vi "VHistFile - Read-Write CDB Log File.vi"(4 "time range to read":cluster{"t1":dbl, "t2":dbl} {"t2" format="%<%H:%M:%S%2u\n%d/%m/%Y>T"; "t1" format="%<%H:%M:%S%2u\n%d/%m/%Y>T"}, 5 "file params":T1={"path pattern"=enum."Y\\M\\D\\Tag.ext", "file extension (.bin)"=".bin"}, 6 "operation":enum16{"nop", "read", "write", "retrieve"}(ring), 7 "log directory":path=path "DataLog", 8 "error in":errorcluster, 9 "history data in":cdb[](array[numeric]) format="%.2f", 10 "time stamps in":dbl[](array[numeric]) format="%<%H:%M:%S%2u\n%d/%m/%Y>T", 11 "file tag":string) -> (0 "error out":errorcluster, 1 "history data out":cdb[](array[numeric]) format="%.2f", 2 "time stamps out":dbl[](array[numeric]) format="%<%H:%M:%S%2u\n%d/%m/%Y>T")   [LabVIEW 2021]
doc: "The VI writes and reads log files intended to store historical data that have <b>CDB Scalar</b> datatype.\n\nA log file record consists of a time stamp and respective data value. VI maintains a separate file for every date; i.e. data values stored in a log file have time stamps belonging to the same date. In addition, VI supports a few file path patterns that define a structure of subdirectories within a basic log directory to store log files and file name format.\n\nVI performs all operations to maintain this file arrangement transparently for applications. An application has only to specify a <b>file tag</b> that is used as a unique data identifier and, optionally, file path pattern and a file name extension.\n\nWhen VI writes historic data, it saves data values and time stamps to the respective file(s). If a file exists, VI appends new records to the end of file. If a file does not exist, VI automatically creates it along with a subdirectory structure it should reside. If an input data set contains values belonging to different dates, VI stores every value to an appropriate location.\n\nWhen VI reads historic data, it automatically retrieves data with time stamps belonging to the specified time range even if required data are stored in several files and, probably, directories. The only required thing is to provide the same file parameters for reading as were used for writing; i.e. file tag, basic log directory, file path pattern and file extension.\n\n::: CalcExpress Toolkit :::\nCopyright (c) 2000-2026 Konstantin Shifershteyn. All rights reserved."
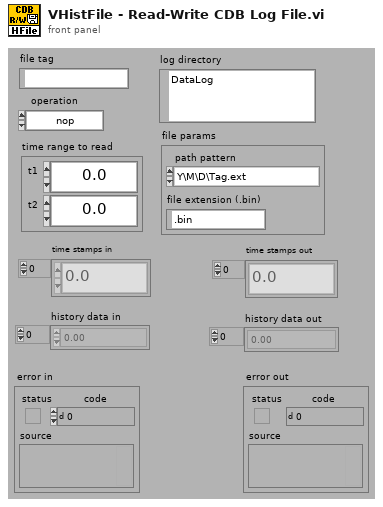
[diagram p1: front panel]
types:
  T1 = cluster{"path pattern":enum32{"Y\\M\\D\\Tag.ext", "Y\\M\\D\\Tag [Y-M-D].ext", "Y-M-D\\Tag.ext", "Y-M-D\\Tag [Y-M-D].ext", "Tag [Y-M-D].ext"}, "file extension (.bin)":string}
  T2 = enum32{"Y\\M\\D\\Tag.ext", "Y\\M\\D\\Tag [Y-M-D].ext", "Y-M-D\\Tag.ext", "Y-M-D\\Tag [Y-M-D].ext", "Tag [Y-M-D].ext"}
  T3 = enum16{"read/write", "read-only", "write-only", "write-only (truncate)"}
  T4 = enum16{"big-endian, network order", "native, host order", "little-endian"}
  T5 = enum16{"deny read/write", "deny write-only", "deny none"}
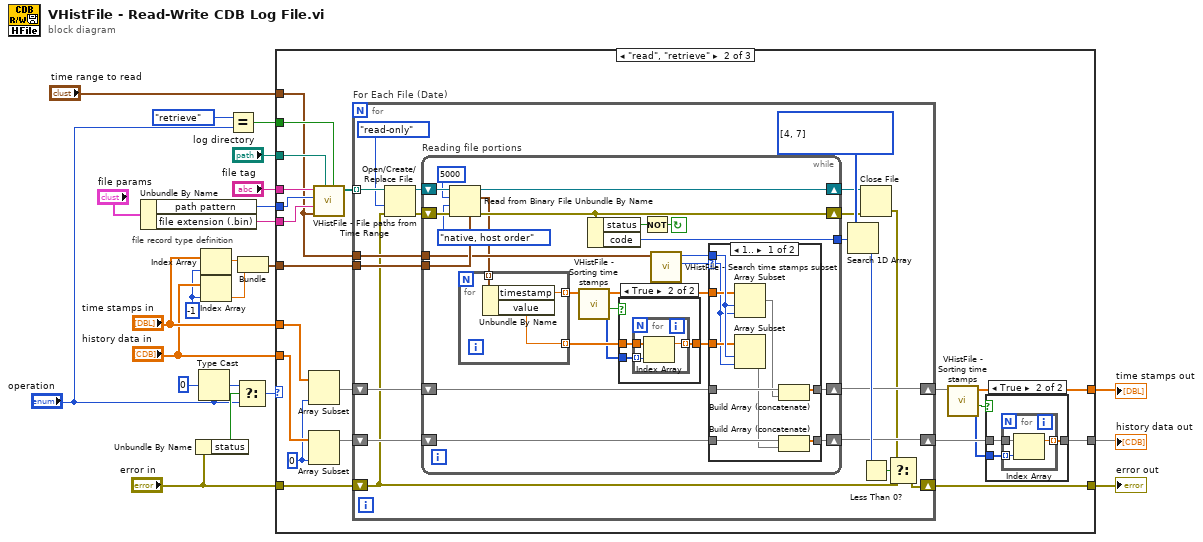
[diagram p0: block diagram]
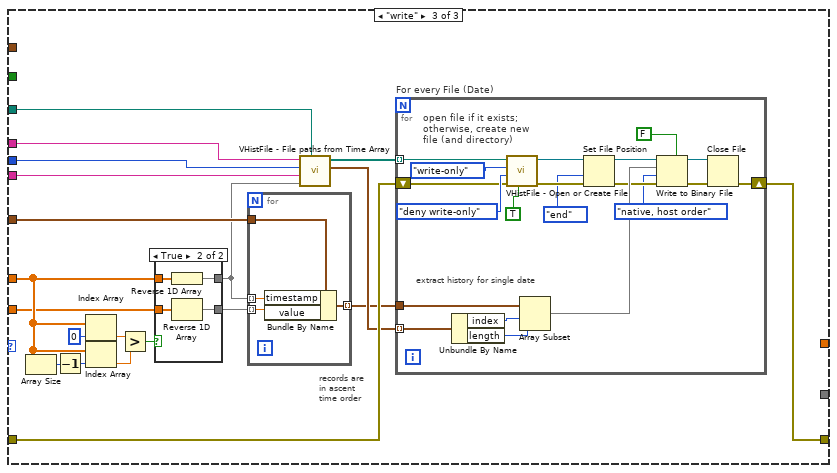
[diagram p6: hidden frame]
diagram:
  w10 = -1
  # "file record type definition"
  n1 = Unbundle By Name("file params") -> ("path pattern"=w14:T2, "file extension (.bin)"=w13:string)
  n2 = Unbundle By Name("error in") -> ("status"=w18:bool)
  n3 = Type Cast(type="operation", x=0) -> (*(type *) &x=w16:enum16{"nop", "read", "write", "retrieve"})
  n4 = Index Array(array="time stamps in", index=w10) -> (element=w9:dbl)
  n5 = Index Array(array="history data in", index=w10) -> (element=w8:cdb)
  n6 = Equal?(x=enum16{"nop", "read", "write", "retrieve"}."retrieve", y="operation") -> (x = y?=w6:bool)
  n7 = Select(t=w16, s=w18, f="operation") -> (s? t:f=w19:enum16{"nop", "read", "write", "retrieve"})
  n8 = Bundle("timestamp"=w9, "value"=w8) -> (w7:cluster{"timestamp":dbl, "value":cdb})  [unwired: 1 in]
  n9 = case shown="\"read\", \"retrieve\"" w19 {
    tunnel: "error in" -> [w24 w39 w132]
    tunnel: [w24 w38 w131] -> w23
    tunnel: "file tag" -> [_ w45 w137]
    tunnel: w7 -> [_ w40 w127]
    tunnel: "log directory" -> [_ w43 w130]
    tunnel: w14 -> [_ w37 w121]
    tunnel: w13 -> [_ w36 w120]
    tunnel: "time stamps in" -> [_ w34 w119]
    tunnel: "history data in" -> [_ w33 w118]
    tunnel: w6 -> [_ w28 _]
    tunnel: [_ w27 _] -> w3
    tunnel: [_ w26 _] -> w2
    tunnel: "time range to read" -> [_ w25 _]
    frame "nop" {
    }
    frame "read", "retrieve" {
      w32 = 0
      n10 = Array Subset(array=w34, length=w32) -> (w42:dbl[])  [unwired: 1 in]
      n11 = Array Subset(array=w33, length=w32) -> (w41:cdb[])  [unwired: 1 in]
      n12 = call "VHistFile - File paths from Time Range.vi"("extended range (F)"=w28, "log directory"=w43, "time range"=w25, "file extension (.bin)"=w36, "path pattern"=w37, "file tag"=w45) -> ("file paths"=w44:path[])  [unwired: 3 in]
      n13 = for "For Each File (Date)" {
        tunnel: w44 -> [w71] mode=indexing
        shift-right: [w57] -> w30
        shift-left: w42 -> [w60]
        tunnel: w40 -> [w70]
        tunnel: w25 -> [w58]
        shift-right: [w56] -> w35
        shift-left: w41 -> [w59]
        shift-right: [w65] -> w38
        shift-left: w39 -> [w55]
        w68 = u16[] [4, 7] items=["No error", "Argument error", "Memory is full", "Out of zone", "End of file", "File already open", "Generic file I/O error", "File not found", "File permission error", "Disk is full", "Duplicate path", "Too many files open", "System feature not enabled", "Resource file not found", "Cannot add resource", "Resource not found", "Image not found", "Image memory error", "Pen does not exist", "Config type invalid", "Config token not found", "Config parse error", "Config memory error", "Bad external code format", "Bad external code offset", "External code not present", "Null window", "Destroy window error", "Null menu", "Print aborted", "Bad print record", "Print driver error", "Windows error during printing", "Memory error during printing", "Print dialog error", "Generic print error", "Invalid device refnum", "Device not found", "Device parameter error", "Device unit error", "Cannot open device", "Device call aborted", "Generic error", "Cancelled by user", "Object ID too low", "Object ID too high", "Object not in heap", "Unknown heap", "Unknown object (invalid DefProc)", "Unknown object (DefProc not in table)", "Message out of range", "Invalid (null) method", "Unknown message", "Manager call not supported", "Bad address", "Network operation in progress", "Network operation timed out", "Connection is busy", "Network attribute not supported", "Network error", "Address in use", "System out of memory", "Connection aborted", "Connection refused", "Not connected", "Already connected", "Connection closed", "Initialization error (interapplication manager)", "Bad occurrence", "Wait on unbound occurrence handler", "Occurrence queue overflow", "Datalog type conflict", "Unused", "Unrecognized type (interapplication manager)", "Memory corrupt", "Failed to make temporary DLL", "Old CIN version", "Drag socket not found", "Failed to load drop-object", "Failed to register OLE object", "Failed to release OLE object", "Format specifier type mismatch", "Unknown format specifier", "Too few format specifiers", "Too many format specifiers", "Scan failed", "Newer CIN version", "OLE Convert", "Runtime menu error", "Password tampered", "Unknown error code"]
        n14 = Open/Create/Replace File ("Open File")(file path (use dialog)=w71, error in=w55, access (0:read/write)=T3."read-only" ("open mode (0)")) -> (refnum out=w64:refnum<file>, error out=w63:errorcluster)  [unwired: 3 in, 1 out]
        n15 = while "Reading file portions" {
          tunnel: [w83] -> w53
          tunnel: w58 -> [w80]
          shift-left: w59 -> [w86]
          shift-right: [w84] -> w56
          shift-left: w60 -> [w87]
          shift-right: [w85] -> w57
          shift-left: w64 -> [w93]
          shift-right: [w92] -> w61
          shift-left: w63 -> [w94]
          shift-right: [w89] -> w62
          tunnel: w70 -> [w95]
          stop <- w88 continue-if-true
          n16 = Read from Binary File ("Read File")(5:w95, 8:w94, 9:T4."native, host order" ("byte order (0:big-endian, network order)"), 10:5000 ("count"), 11:w93) -> (0:w89:errorcluster, 2:w79:cluster{"timestamp":dbl, "value":cdb}[], 3:w92:refnum<file>)  [unwired: 1 in, 1 out]
          n17 = for {
            tunnel: [w117] -> w78 mode=indexing
            tunnel: [w116] -> w77 mode=indexing
            tunnel: w79 -> [w115] mode=indexing
            n18 = Unbundle By Name(w115) -> ("timestamp"=w117:dbl, "value"=w116:cdb)
          }
          n19 = call "VHistFile - Sorting time stamps.vi"("time stamps in"=w78) -> ("indexes out"=w75:i32[], "sorted"=w73:bool, "time stamps out"=w74:dbl[])  [unwired: 6 in]
          n20 = Unbundle By Name(w89) -> ("status"=w90:bool, "code"=w83:i32)
          n21 = case shown="True" w73 {
            tunnel: w77 -> [w96 w99]
            tunnel: [w96 w98] -> w76
            tunnel: w75 -> [_ w97]
            frame False {
            }
            frame True {
              n22 = for {
                tunnel: w99 -> [w102]
                tunnel: [w101] -> w98 mode=indexing
                tunnel: w97 -> [w100] mode=indexing
                n23 = Index Array(array=w102, index=w100) -> (element=w101:cdb)
              }
            }
          }
          n24 = Not(x=w90) -> (.not. x?=w88:bool)
          n25 = call "VHistFile - Search time stamps subset.vi"("time stamps"=w74, "time range"=w80) -> ("length"=w81:i32, "index"=w82:i32)  [unwired: 6 in]
          n26 = case shown="1.." w81 {
            selector: w81 -> [w103 _]
            tunnel: w82 -> [w112 _]
            tunnel: w74 -> [w111 _]
            tunnel: w76 -> [w110 _]
            tunnel: w87 -> [w109 w114]
            tunnel: w86 -> [w108 w113]
            tunnel: [w107 w114] -> w85
            tunnel: [w104 w113] -> w84
            frame 1.. {
              n27 = Array Subset(array=w111, index=w112, length=w103) -> (w106:dbl[])
              n28 = Array Subset(array=w110, index=w112, length=w103) -> (w105:cdb[])
              n29 = Build Array (concatenate)(w109, w106) -> (w107:dbl[])
              n30 = Build Array (concatenate)(w108, w105) -> (w104:cdb[])
            }
            frame ..0 {
            }
          }
        }
        n31 = Search 1D Array(1D array=w68, element=w53) -> (index of element=w66:i32)  [unwired: 1 in]
        n32 = Close File(refnum=w61, error in=w62) -> (error out=w54:errorcluster)  [unwired: 1 out]
        n33 = Less Than 0?(x=w66) -> (x < 0?=w67:bool)
        n34 = Select(t=w54, s=w67, f=w55) -> (s? t:f=w65:errorcluster)
      }
      n35 = call "VHistFile - Sorting time stamps.vi"("time stamps in"=w30) -> ("indexes out"=w31:i32[], "sorted"=w29:bool, "time stamps out"=w26:dbl[])  [unwired: 6 in]
      n36 = case shown="True" w29 {
        tunnel: w35 -> [w46 w49]
        tunnel: [w46 w48] -> w27
        tunnel: w31 -> [_ w47]
        frame False {
        }
        frame True {
          n37 = for {
            tunnel: w49 -> [w52]
            tunnel: [w51] -> w48 mode=indexing
            tunnel: w47 -> [w50] mode=indexing
            n38 = Index Array(array=w52, index=w50) -> (element=w51:cdb)
          }
        }
      }
    }
    frame "write" {
      # "records are\nin ascent\ntime order"
      n39 = Array Size(array=w119) -> (size(s)=w135:i32)
      n40 = Decrement(x=w135) -> (x-1=w134:i32)
      n41 = Index Array(array=w119, index=0) -> (element=w126:dbl)
      n42 = Index Array(array=w119, index=w134) -> (element=w125:dbl)
      n43 = Greater?(x=w126, y=w125) -> (0:w133:bool)
      n44 = case shown="True" w133 {
        tunnel: w118 -> [w159 w163]
        tunnel: [w159 w162] -> w128
        tunnel: w119 -> [w158 w161]
        tunnel: [w158 w160] -> w122
        frame False {
        }
        frame True {
          n45 = Reverse 1D Array(array=w161) -> (reversed array=w160:dbl[])
          n46 = Reverse 1D Array(array=w163) -> (reversed array=w162:cdb[])
        }
      }
      n47 = for {
        tunnel: w128 -> [w166] mode=indexing
        tunnel: [w167] -> w123 mode=indexing
        tunnel: w127 -> [w164]
        tunnel: w122 -> [w165] mode=indexing
        n48 = Bundle By Name(cluster=w164, "timestamp"=w165, "value"=w166) -> (w167:cluster{"timestamp":dbl, "value":cdb})
      }
      n49 = call "VHistFile - File paths from Time Array.vi"("log directory"=w130, "time stamps"=w122, "file extension (.bin)"=w120, "path pattern"=w121, "file tag"=w137) -> ("subset info"=w124:cluster{"index":i32, "length":i32}[], "file paths"=w129:path[])  [unwired: 3 in]
      n50 = for "For every File (Date)" {
        tunnel: w129 -> [w154] mode=indexing
        shift-right: [w148] -> w131
        shift-left: w132 -> [w149]
        tunnel: w124 -> [w146] mode=indexing
        tunnel: w123 -> [w142]
        # "open file if it exists;\notherwise, create new\nfile (and directory)"
        # "extract history for single date"
        n51 = Unbundle By Name(w146) -> ("index"=w145:i32, "length"=w144:i32)
        n52 = call "VHistFile - Open or Create File.vi"("create if doesn't exist (F)"=TRUE, "error in"=w149, "deny mode (2)"=T5."deny write-only", "open mode (0)"=T3."write-only", "file path"=w154) -> ("error out"=w151:errorcluster, "file refnum"=w155:refnum<file>)  [unwired: 5 in]
        n53 = Array Subset(array=w142, index=w145, length=w144) -> (w143:cluster{"timestamp":dbl, "value":cdb}[])
        n54 = Set File Position(refnum=w155, from (0:start)=enum16{"start", "end", "current"}."end" ("pos mode (0:2)"), error in=w151) -> (refnum out=w141:refnum<file>, error out=w140:errorcluster)  [unwired: 1 in]
        n55 = Write to Binary File ("Write File")(file (use dialog)=w141, data=w143, error in=w140, 5:FALSE ("prepend array or string size? (T)"), 9:T4."native, host order" ("byte order (0:big-endian, network order)")) -> (refnum out=w156:refnum<file>, error out=w157:errorcluster)  [unwired: 1 in, 1 out]
        n56 = Close File(refnum=w156, error in=w157) -> (error out=w148:errorcluster)  [unwired: 1 out]
      }
    }
  }
  "error out" <- w23
  "history data out" <- w3
  "time stamps out" <- w2
